vi "py2vi.vi"   [LabVIEW 2026]
doc: "Launcher for g-cli. This VI parses cli arguments, sets up the required interfaces and runs the process through the Runner Actor."
uses:
  <vilib>/ActorFramework/Actor/Actor.lvclass
  Actors/Runner/Runner/Runner.lvclass
  Actors/Runner/Runner/Runner.lvclass/Runner.ctl
  Actors/Console Logger/Console Logger/Console Logger.lvclass
  Actors/Console Logger/Console Logger/Console Logger.lvclass/Console Logger.ctl
  Actors/File Logger/File Logger/File Logger.lvclass
  Actors/File Logger/File Logger/File Logger.lvclass/File Logger.ctl
  Interfaces/ILogger Client/ILogger Client Messages/Set Logger Enqueuer Msg/Set Logger Enqueuer Msg.lvclass/Set Logger Enqueuer Msg.ctl
  <vilib>/ActorFramework/Message Enqueuer/Message Enqueuer.lvclass/Message Enqueuer.ctl
  Interfaces/IRunner/IRunner Messages/Set Interfaces Msg/Set Interfaces Msg.lvclass/Set Interfaces Msg.ctl
  Interfaces/IRunner/IRunner Messages/Run Msg/Run Msg.lvclass/Run Msg.ctl
  <vilib>/ActorFramework/Stop Msg/Stop Msg.lvclass/Stop Msg.ctl
  Actors/Console Logger/Console Logger/Write CLI Reference.vi
  Actors/File Logger/File Logger/Write Log File.vi
  Actors/Runner/Runner/Write Stop Event.vi
  <vilib>/ActorFramework/Message Enqueuer/Enqueue Critical.vi
  <vilib>/ActorFramework/Message Enqueuer/Enqueue.vi
  Interfaces/ILogger Client/ILogger Client Messages/Set Logger Enqueuer Msg/Set Logger Enqueuer Msg.lvclass
  Interfaces/IRunner/IRunner Messages/Set Interfaces Msg/Set Interfaces Msg.lvclass
  Interfaces/IRunner/IRunner Messages/Run Msg/Run Msg.lvclass
  <vilib>/ActorFramework/Stop Msg/Stop Msg.lvclass
  <vilib>/ActorFramework/Message Priority Queue/Priority Enqueue.vi
  <vilib>/Wiresmith Technology/G CLI/CLI Class/CLI.lvclass
  <vilib>/Wiresmith Technology/G CLI/Argument Parser/Option Set Class/Option Set.lvclass
panel:
  # "py2vi Launcher"
types:
  T1 = typedef "Option Parser.lvlib/Option.lvclass/Option Configuration.ctl" = cluster{"Option Type":T2, "Option Labels":string[], "Key":string, "Description":string, "Required":bool, "Default Value":string}
  T2 = typedef "Option Parser.lvlib/Option.lvclass/Argument Type.ctl" = enum16{"flag", "value"}
  T3 = typedef "IRunner.lvlib/IRunner.lvclass/Interfaces--cluster.ctl" = cluster{"IProject Manager":refnum<class "IProject Manager.lvclass">, "IFile Manager":refnum<class "IFile Manager.lvclass">, "IPython Caller":refnum<class "IPython Caller.lvclass">, "IElement Manager":refnum<class "IElement Manager.lvclass">, "ILV File Creator":refnum<class "ILV File Creator.lvclass">, "IHash Whitelist Handler":refnum<class "IHash Whitelist Handler.lvclass">}
  T4 = typedef "NI_App_Builder_API.lvlib/Build Specification Version.ctl" = cluster{"Major":u16, "Minor":u16, "Fix":u16, "Build":u16}
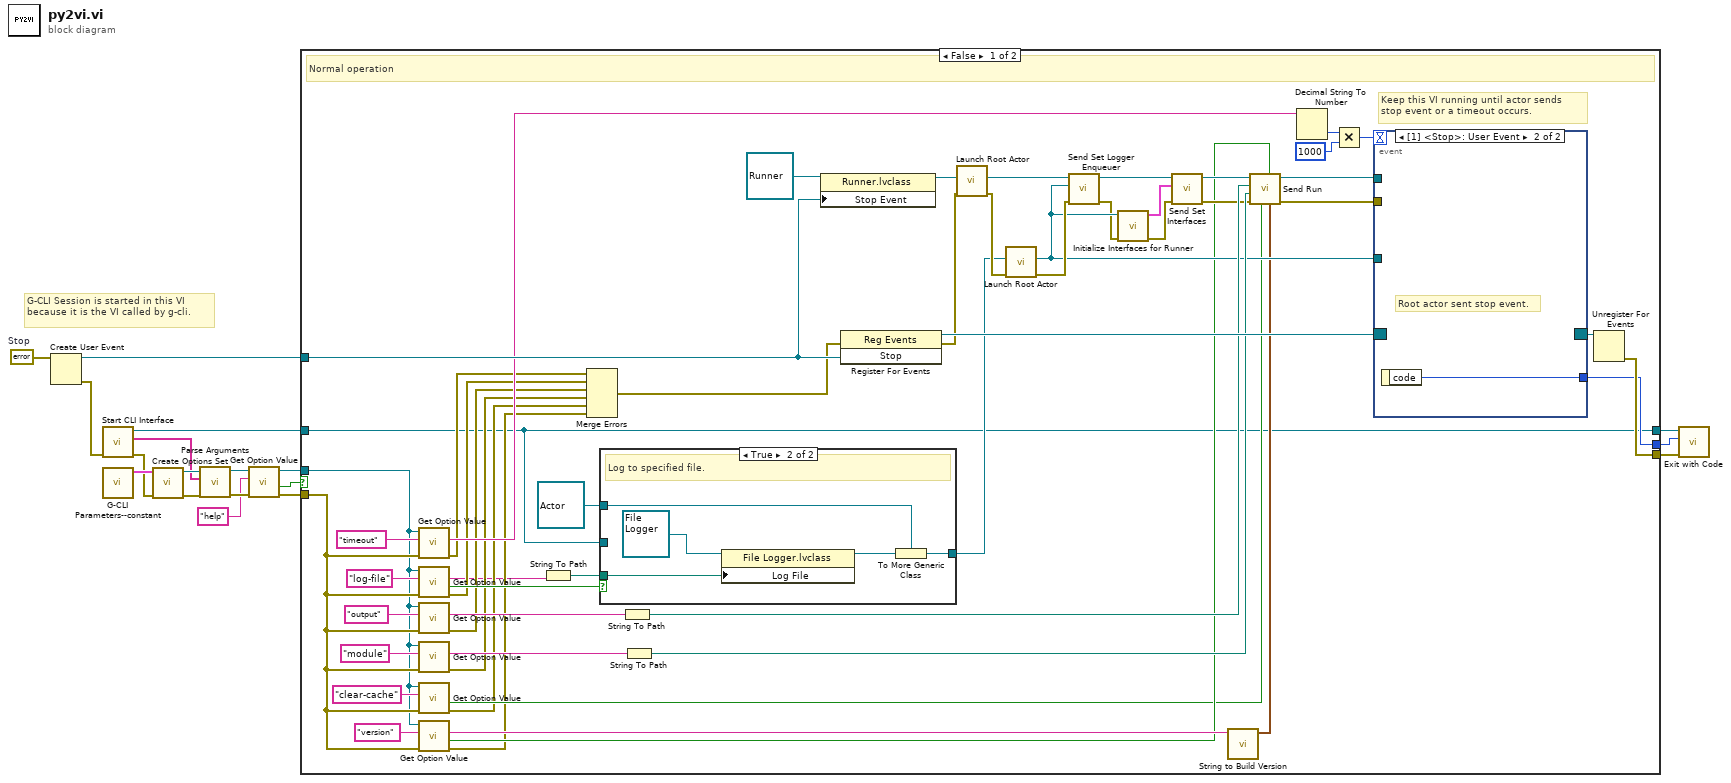
[diagram p0: block diagram]
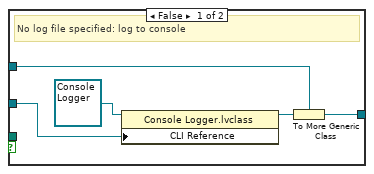
[diagram p2: hidden frame]
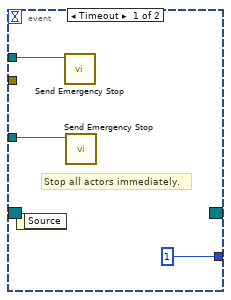
[diagram p3: hidden frame]
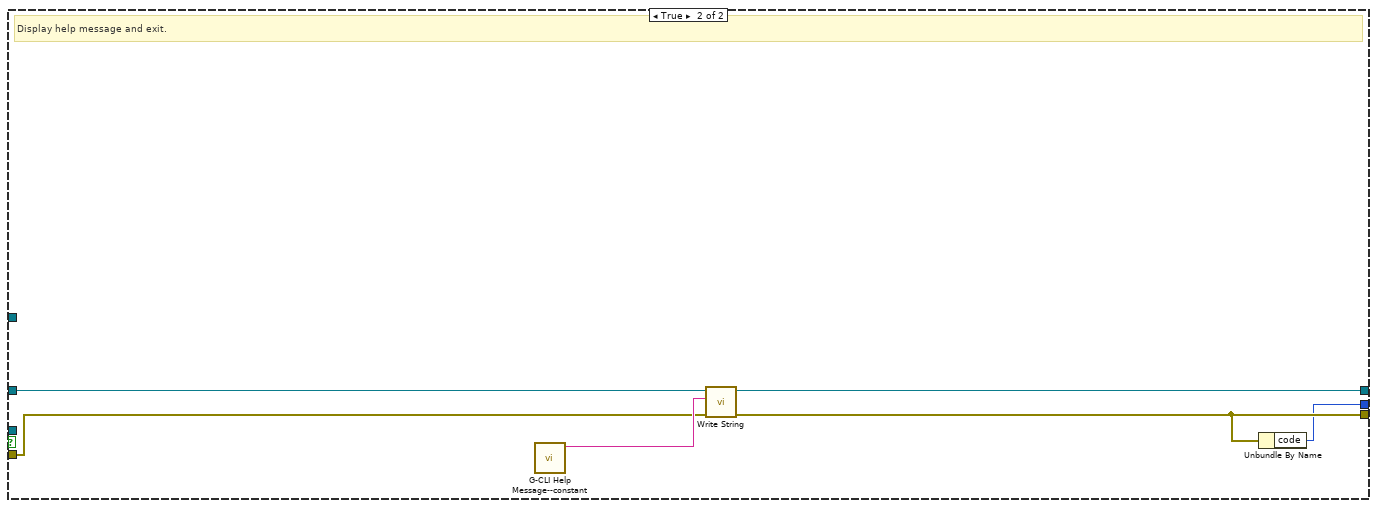
[diagram p4: hidden frame]
diagram:
  w1 = errorcluster {"status"=FALSE, "code"=0, "source"=""}  # Stop
  # "G-CLI Session is started in this VI because it is the VI called by g-cli."
  n1 = Create User Event(user event datatype=w1) -> (user event=w17:refnum<user-event>, error out=w18:errorcluster)  [unwired: 1 in]
  n2 = call <vilib>:"Start CLI Interface.vi"("error in (no error)"=w18) -> ("error out"=w12:errorcluster, "Custom Parameters"=w14:string[], "CLI out"=w9:refnum<class "CLI.lvclass">)  [unwired: 7 in, 1 out]
  n3 = call "G-CLI Parameters--constant.vi"() -> ("G-CLI Parameters"=w13:T1[])  [unwired: 11 in]
  n4 = call <vilib>:"Create Options Set.vi"("error in (no error)"=w12, "Options"=w13) -> ("error out"=w15:errorcluster, "Option Set out"=w16:refnum<class "Option Set.lvclass">)  [unwired: 8 in]
  n5 = call <vilib>:"Parse Arguments.vi"("error in (no error)"=w15, "Arguments"=w14, "Option Set in"=w16) -> ("error out"=w6:errorcluster, "Option Set out"=w8:refnum<class "Option Set.lvclass">)  [unwired: 5 in, 2 out]
  n6 = call <vilib>:"Get Option Value.vi"("error in (no error)"=w6, "Option Key"="help", "Option Set in"=w8) -> ("error out"=w5:errorcluster, "Set"=w3:bool, "Option Set out"=w7:refnum<class "Option Set.lvclass">)  [unwired: 5 in, 1 out]
  n7 = case shown="False" w3 {
    tunnel: w17 -> [w70 _]
    tunnel: [w35 w87] -> w11
    tunnel: [w34 w86] -> w10
    tunnel: w9 -> [w19 w91]
    tunnel: w5 -> [w30 w88]
    tunnel: w7 -> [w29 _]
    tunnel: [w19 w90] -> w2
    frame False {
      # "Keep this VI running until actor sends stop event or a timeout occurs."
      # "Normal operation"
      n8 = call <vilib>:"Get Option Value.vi"("error in (no error)"=w30, "Option Key"="timeout", "Option Set in"=w29) -> ("error out"=w23:errorcluster, "Value"=w62:string)  [unwired: 5 in, 2 out]
      n9 = call <vilib>:"Get Option Value.vi"("error in (no error)"=w30, "Option Key"="log-file", "Option Set in"=w29) -> ("error out"=w24:errorcluster, "Set"=w33:bool, "Value"=w21:string)  [unwired: 5 in, 1 out]
      n10 = call <vilib>:"Get Option Value.vi"("error in (no error)"=w30, "Option Key"="output", "Option Set in"=w29) -> ("error out"=w25:errorcluster, "Value"=w65:string)  [unwired: 5 in, 2 out]
      n11 = call <vilib>:"Get Option Value.vi"("error in (no error)"=w30, "Option Key"="module", "Option Set in"=w29) -> ("error out"=w26:errorcluster, "Value"=w64:string)  [unwired: 5 in, 2 out]
      n12 = call <vilib>:"Get Option Value.vi"("error in (no error)"=w30, "Option Key"="clear-cache", "Option Set in"=w29) -> ("error out"=w27:errorcluster, "Set"=w37:bool)  [unwired: 5 in, 2 out]
      n13 = call <vilib>:"Get Option Value.vi"("error in (no error)"=w30, "Option Key"="version", "Option Set in"=w29) -> ("error out"=w28:errorcluster, "Set"=w39:bool, "Value"=w46:string)  [unwired: 5 in, 1 out]
      n14 = String To Path(string=w21) -> (path=w20:path)
      n15 = Merge Errors(w23, w24, w25, w26, w27, w28) -> (w22:errorcluster)
      n16 = case shown="True" w33 {
        tunnel: w19 -> [w75 _]
        tunnel: refnum<class "Actor.lvclass"> refnum ("Actor") -> [w74 w81]
        tunnel: [w72 w78] -> w31
        tunnel: w20 -> [_ w77]
        frame False {
          # "No log file specified: log to console"
          n17 = property class="Console Logger.lvclass"(reference=refnum<class "Console Logger.lvclass"> refnum ("Console Logger.lvlib:Console Logger.lvclass"), "CLI Reference"=w75) -> (reference out=w73:refnum<class "Console Logger.lvclass">)  [unwired: 1 in, 1 out]
          n18 = To More Generic Class(target class=w74, reference=w73) -> (generic class reference=w72:refnum<class "Actor.lvclass">)
        }
        frame True {
          # "Log to specified file."
          n19 = property class="File Logger.lvclass"(reference=refnum<class "File Logger.lvclass"> refnum ("File Logger.lvlib:File Logger.lvclass"), "Log File"=w77) -> (reference out=w79:refnum<class "File Logger.lvclass">)  [unwired: 1 in, 1 out]
          n20 = To More Generic Class(target class=w81, reference=w79) -> (generic class reference=w78:refnum<class "Actor.lvclass">)
        }
      }
      n21 = String To Path(string=w65) -> (path=w56:path)
      n22 = String To Path(string=w64) -> (path=w55:path)
      n23 = property class="Runner.lvclass"(reference=refnum<class "Runner.lvclass"> refnum ("G-CLI Runner.lvlib:G-CLI Runner.lvclass"), "Stop Event"=w70) -> (reference out=w58:refnum<class "Runner.lvclass">)  [unwired: 1 in, 1 out]
      n24 = register-events(error in=w22, w70) -> (reference out=w69:refnum<event-registration>, error out=w48:errorcluster)  [unwired: 1 in]
      n25 = call <vilib>:"Launch Root Actor.vi"("error in (no error)"=w48, "Actor"=w58) -> ("error out"=w51:errorcluster, "Actor's Enqueuer"=w52:refnum<class "Message Enqueuer.lvclass">)  [unwired: 8 in]
      n26 = call <vilib>:"Launch Root Actor.vi"("error in (no error)"=w51, "Actor"=w31) -> ("error out"=w57:errorcluster, "Actor's Enqueuer"=w45:refnum<class "Message Enqueuer.lvclass">)  [unwired: 8 in]
      n27 = call "Send Set Logger Enqueuer.vi"("error in (no error)"=w57, "Logger"=w45, "Message Enqueuer"=w52) -> ("error out"=w44:errorcluster, "Message Enqueuer out"=w42:refnum<class "Message Enqueuer.lvclass">)  [unwired: 7 in]
      n28 = call "Initialize Interfaces for Runner.vi"("error in"=w44, "Logger Enqueuer"=w45) -> ("error out"=w41:errorcluster, "Interfaces"=w43:T3)  [unwired: 8 in]
      n29 = call "Send Set Interfaces.vi"("error in (no error)"=w41, "Interfaces"=w43, "Message Enqueuer"=w42) -> ("error out"=w49:errorcluster, "Message Enqueuer out"=w50:refnum<class "Message Enqueuer.lvclass">)  [unwired: 7 in]
      n30 = call "String to Build Version.vi"("Version String"=w46) -> ("Build Specification Version"=w40:T4)  [unwired: 9 in, 1 out]
      n31 = call "Send Run.vi"("Build Specification Version"=w40, "Set PPL Version"=w39, "Clear Compiled Object Cache"=w37, "error in (no error)"=w49, "Python Module"=w55, "Output Folder"=w56, "Message Enqueuer"=w50) -> ("error out"=w53:errorcluster, "Message Enqueuer out"=w54:refnum<class "Message Enqueuer.lvclass">)  [unwired: 3 in]
      n32 = Decimal String To Number(string=w62) -> (number=w61:i32)  [unwired: 2 in, 1 out]
      n33 = Multiply(x=w61, y=1000) -> (x*y=w59:i32)
      n34 = event shown="[1] <Stop>: User Event" {
        selector: w69 -> [_ _]
        dyn-events: [_ _] -> w68
        timeout: w59 -> [_ _]
        tunnel: w54 -> [w84 _]
        tunnel: w45 -> [w83 _]
        tunnel: w53 -> [_ _]
        tunnel: [1 w85] -> w34
        event Timeout {
          # "Stop all actors immediately."
          n35 = event-data() -> ()  [unwired: 1 in, 1 out]
          n36 = call <vilib>:"Send Emergency Stop.vi"("Message Enqueuer"=w84) -> ()  [unwired: 10 in, 1 out]
          n37 = call <vilib>:"Send Emergency Stop.vi"("Message Enqueuer"=w83) -> ()  [unwired: 10 in, 1 out]
        }
        event User Event {
          # "Root actor sent stop event."
          n38 = event-data() -> ("code"=w85:i32)  [unwired: 1 in]
        }
      }
      n39 = Unregister For Events(event registration refnum=w68) -> (error out=w35:errorcluster)  [unwired: 1 in]
    }
    frame True {
      # "Display help message and exit."
      n40 = call "G-CLI Help Message--constant.vi"() -> ("G-CLI Help Message"=w89:string)  [unwired: 11 in]
      n41 = call <vilib>:"Write String.vi"("error in (no error)"=w88, "Text to Write"=w89, "CLI in"=w91) -> ("error out"=w87:errorcluster, "CLI out"=w90:refnum<class "CLI.lvclass">)  [unwired: 7 in]
      n42 = Unbundle By Name(w87) -> ("code"=w86:i32)
    }
  }
  n43 = call <vilib>:"Exit with Code.vi"("error in (no error)"=w11, "Exit Code (0)"=w10, "CLI in"=w2) -> ()  [unwired: 8 in, 1 out]
